vi "http.vi"() -> ()   [LabVIEW 2019]
uses:
  <vilib>/httpClient/LabVIEWHTTPClient.lvlib
panel:
  out "body":string
  in  "WebBrowser":refnum<k7>(container)
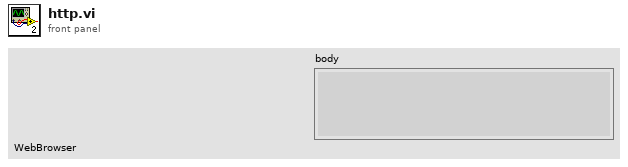
[diagram p1: front panel]
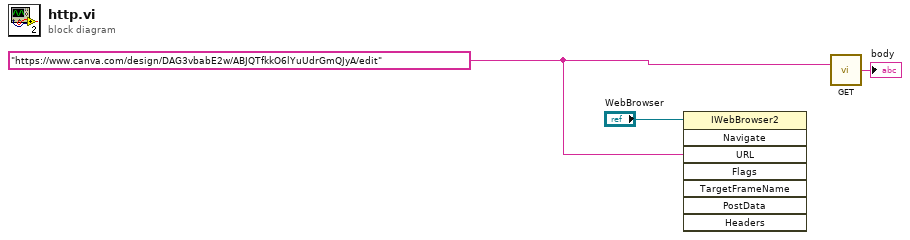
[diagram p0: block diagram]
diagram:
  w2 = "https://www.canva.com/design/DAG3vbabE2w/ABJQTfkkO6lYuUdrGmQJyA/edit" ("url")
  n1 = invoke class="IWebBrowser2" method="Navigate"(reference="WebBrowser", "URL"=w2) -> ()  [unwired: 6 in, 8 out]
  n2 = call <vilib>:"GET.vi"("url"=w2) -> ("body"=→"body":string)  [unwired: 11 in, 3 out]
